vi "test_image_content.vi"(8 "error in":errorcluster) -> (0 "error out":errorcluster, 3 "image":picture)   [LabVIEW 2020, in "Conformance MCP Server.lvlib"]
doc: "Conformance fixture (scenario tools-call-image). Takes no arguments and returns a small red square as a picture; the server sends it as image content (PNG, base64)."
uses:
  Conformance MCP Server.lvlib
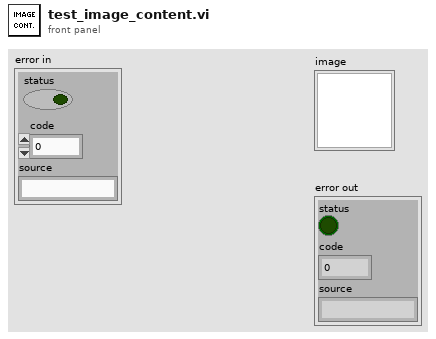
[diagram p1: front panel]
types:
  T1 = cluster{"left":i16, "top":i16, "right":i16, "bottom":i16}
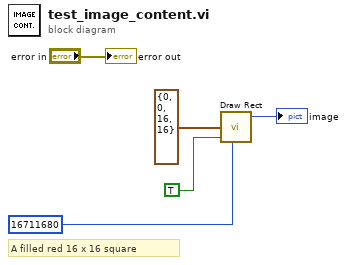
[diagram p0: block diagram]
diagram:
  # "A filled red 16 x 16 square"
  n1 = call <vilib>:"Draw Rect.vi"("rect"=T1 {"left"=0, "top"=0, "right"=16, "bottom"=16}, "fill?(F)"=TRUE, "color(black)"=u32 16711680) -> ("new picture"=→"image":picture)  [unwired: 6 in]
  "error out" <- "error in"
